vi "CommonVIs_ClassWireSelection.vi"(3 "Offset(-300,0)":T1={"Left"=-236, "Top"=18}, 4 "SaveChangesInClassRightAway(True)":bool=TRUE, 5 "WireStyleSelected":refnum<user-event>, 7 "SelectedWireStyle":refnum<vi>, 8 "error in (no error)":errorcluster, 9 "Messages(Stop or Empty string will stop this VI)":refnum<user-event>, 10 "WireSelectionList":refnum<vi>, 11 "LVClassToActOn":refnum<vi>) -> (0 "error out":errorcluster)   [LabVIEW 2020]
uses:
  Provider_BaseClassInterface/BaseProvider_SubVIs/BaseProvider_WireList.ctl
  Provider_BaseClassInterface/BaseProvider_SubVIs/BaseProvider_WireStyleType.ctl
  <vilib>/Utility/miscctls.llb/LVPositionTypeDef.ctl
  SubVIs/GOOP_WireConfigurationType.ctl
  SubVIs/GOOP_WirePattern.ctl
panel:
  out "WireEditorPresses":bool
  out "ListIndexSelected":i32
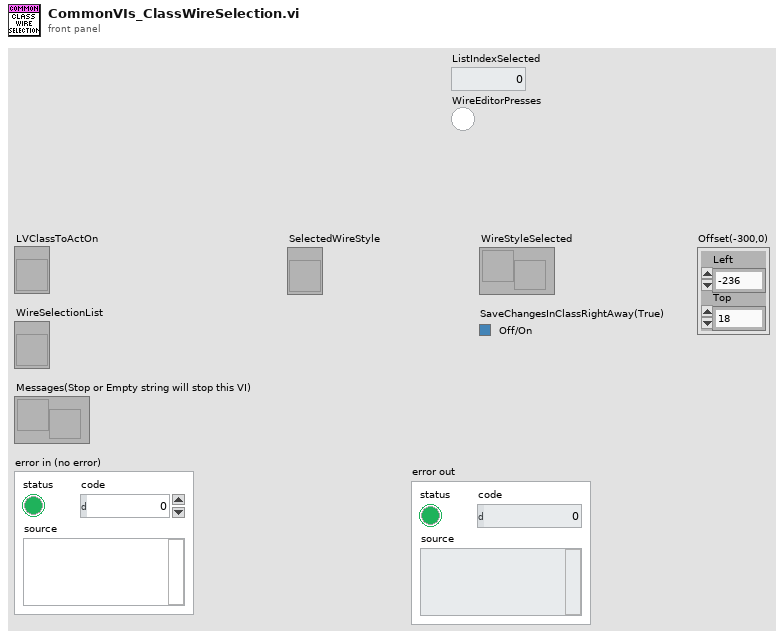
[diagram p1: front panel]
types:
  T1 = typedef "LVPositionTypeDef.ctl" = cluster{"Left":i32, "Top":i32}
  T2 = typedef "GOOP_WireConfigurationType.ctl" = cluster{"Edge thickness":i32, "Edge color":u32, "Center thickness":i32, "Center pattern":T3, "CenterColor1":u32, "CenterColor2":u32, "Tunnels and terminals colors":u32}
  T3 = typedef "GOOP_WirePattern.ctl" = enum16{"Solid", "Large dash", "Small dash"}
  T4 = typedef "BaseProvider_WireList.ctl" = cluster{"WireStyle":T5[], "WireEditor":bool}
  T5 = typedef "BaseProvider_WireStyleType.ctl" = cluster{"Boolean":bool, "Wire":picture, "Name":string, "Status":u16}
  T6 = cluster{"SelectedWireStyle":string, "Timeout":i32, "SelectedWireStyle":T2, "AllWireConfigurations(Names)":string[], "AllWireConfigurations":T2[], "SelectedWireListIndex":i32, "WireSelectionList":T4, "FirstTime":bool, "OverWireListIndex":i32, "MouseDown":bool}
  T7 = cluster{"Foreground Color":u32, "Background Color":u32, "Fill Pattern":cluster{"Row 0":u8, "Row 1":u8, "Row 2":u8, "Row 3":u8, "Row 4":u8, "Row 5":u8, "Row 6":u8, "Row 7":u8}, "Width":i16, "Mode":enum16{"Copy", "Or", "Exclusive Or", "Bit Clear", "Not Copy", "Not Or", "Nor Exclusive Or", "Not Bit Clear"}, "Style":enum32{"Solid", "Dash", "Dot", "Dash Dot", "Dash Dot Dot"}, "Fill Rule":enum32{"Even Odd", "Winding"}, "End Caps":enum32{"Default", "Flat"}}[]
  T8 = typedef "LVBoundsTypeDef.ctl" = cluster{"Width":u32, "Height":u32}
  T9 = typedef "lveventtype.ctl" = enum32{"Null", "Timeout", "Annotation Menu Selection", "Annotation Menu Selection?", "App Instance Close", "App Instance Close?", "Autoscale Range Change", "Bookmark Info Change", "Cell Edit", "Cell Edit?", "Cursor Grab", "Cursor Grab?", "Cursor Menu Selection", "Cursor Menu Selection?", "Cursor Move", "Cursor Release", "Data Change", "Direction Change", "Display State Change", "Drag Ended", "Drag Enter", "Drag Leave", "Drag Over", "Drag Source Update", "Drag Starting", "Drag Starting?", "Drop", "Exec State Change", "Key Down", "Key Down?", "Key Repeat", "Key Repeat?", "Key Up", "Listbox Double Click", "Menu Activation?", "Menu Selection (App)", "Menu Selection? (App)", "Menu Selection (User)", "Mouse Down", "Mouse Down?", "Mouse Enter", "Mouse Leave", "Mouse Move", "Mouse Up", "Mouse Wheel", "NI Security User Change (App)", "Pane Size", "Panel Close", "Panel Close?", "Panel Resize", "Plot Attribute Change", "Scale Range Change", "Shortcut Menu Activation?", "Shortcut Menu Selection (App)", "Shortcut Menu Selection? (App)", "Shortcut Menu Selection (User)", "Tree Double Click", "Tree Drag", "Tree Drag?", "Tree Drop", "Tree Drop?", "Tree Item Close", "Tree Item Close?", "Tree Item Open", "Tree Item Open?", "User Event", "Value Change"}
  T10 = typedef "LVPoint32TypeDef.ctl" = cluster{"Horizontal":i32, "Vertical":i32}
  T11 = cluster{"WireStyle":cluster{"Boolean":bool, "Wire":bool, "Name":bool, "Status":bool}[], "WireEditor":bool}
  T12 = cluster{"Boolean":bool, "Wire":bool, "Name":bool, "Status":bool}[]
  T13 = typedef "Scripting_ConnectorPanePatternType.ctl" = u16
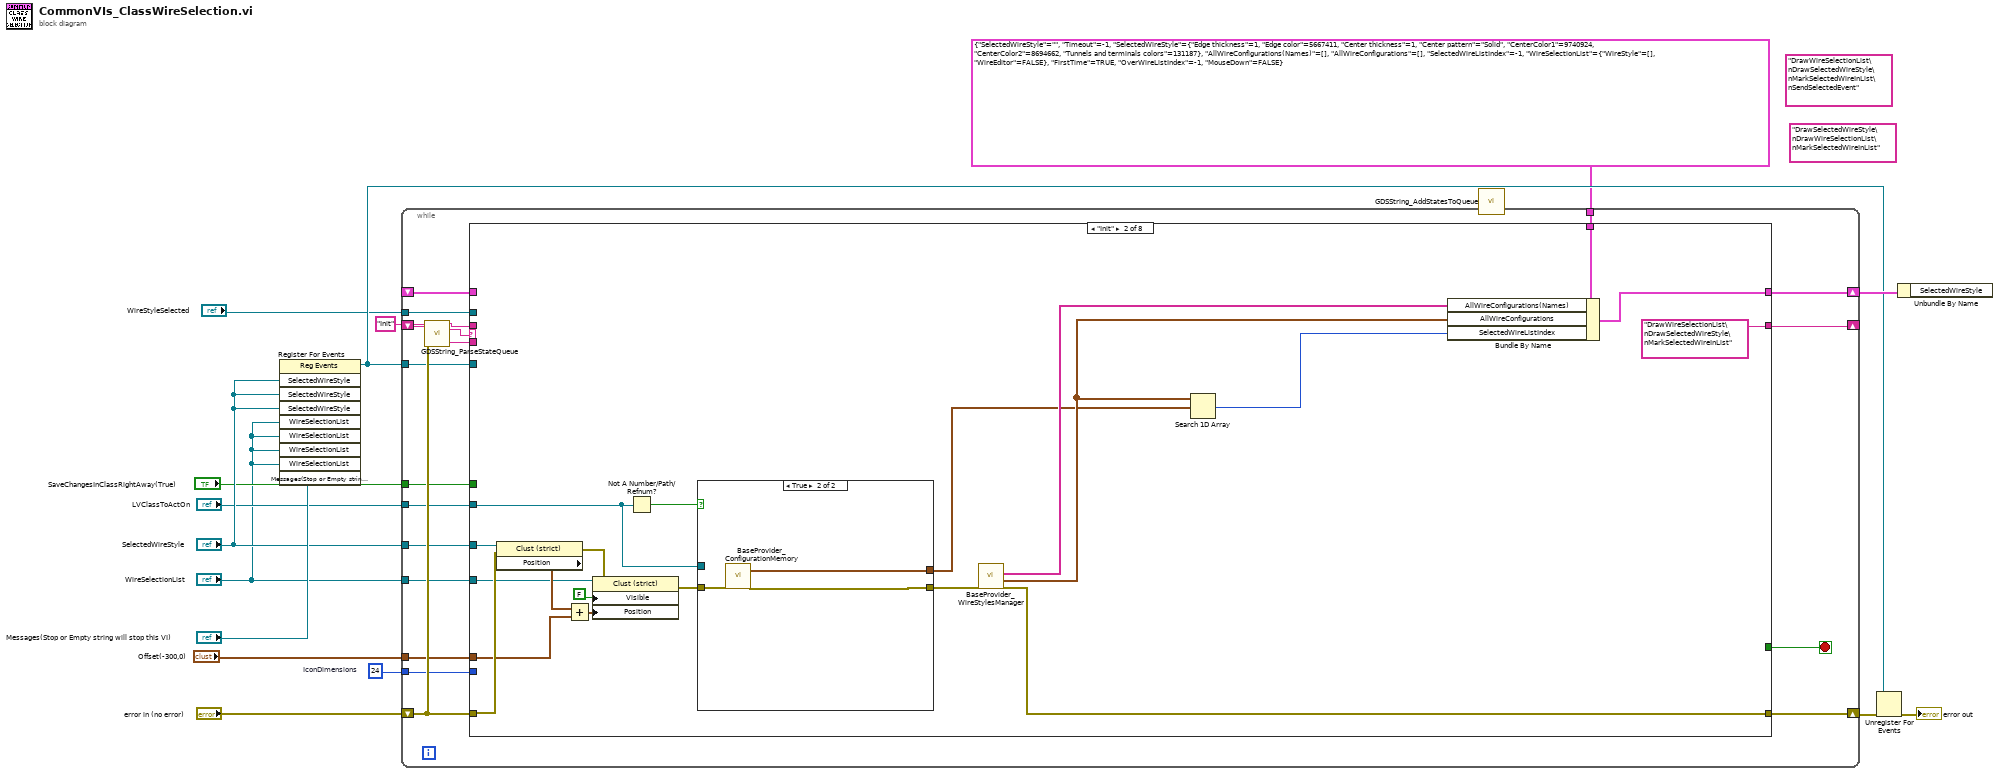
[diagram p0: block diagram]
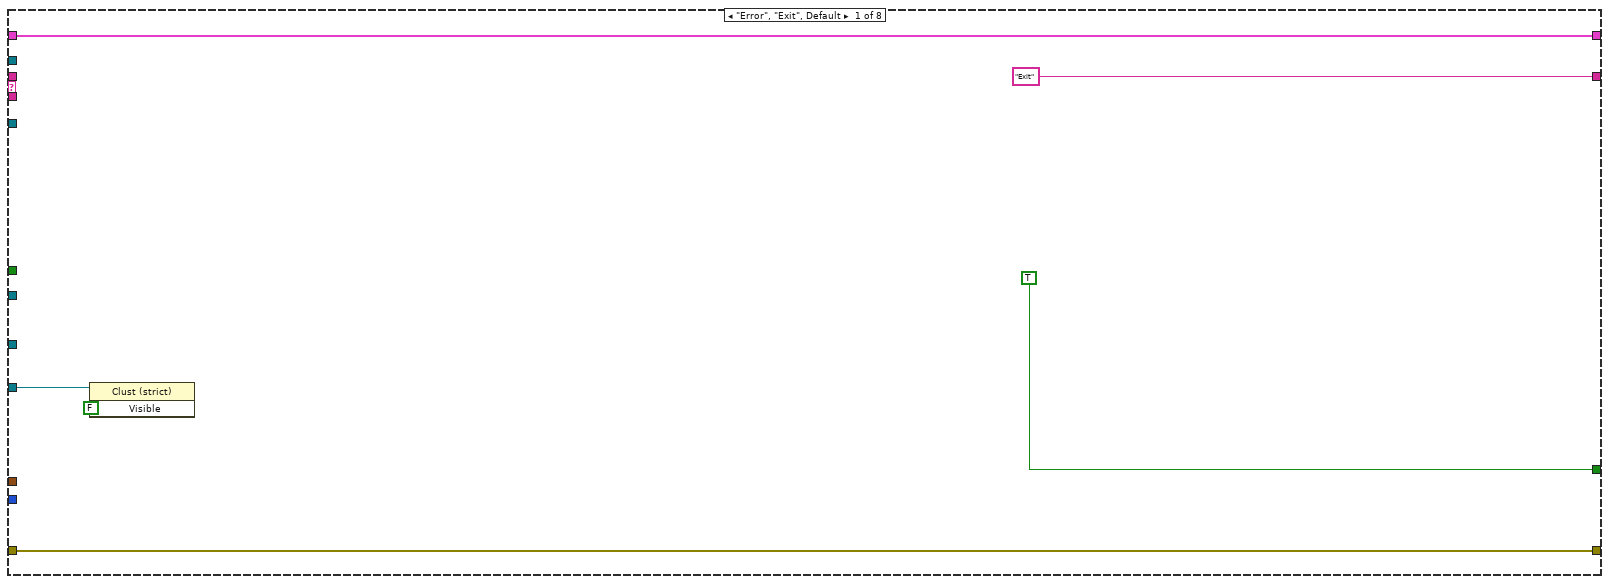
[diagram p2: hidden frame]
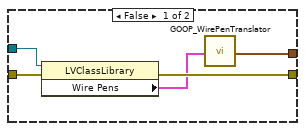
[diagram p3: hidden frame]
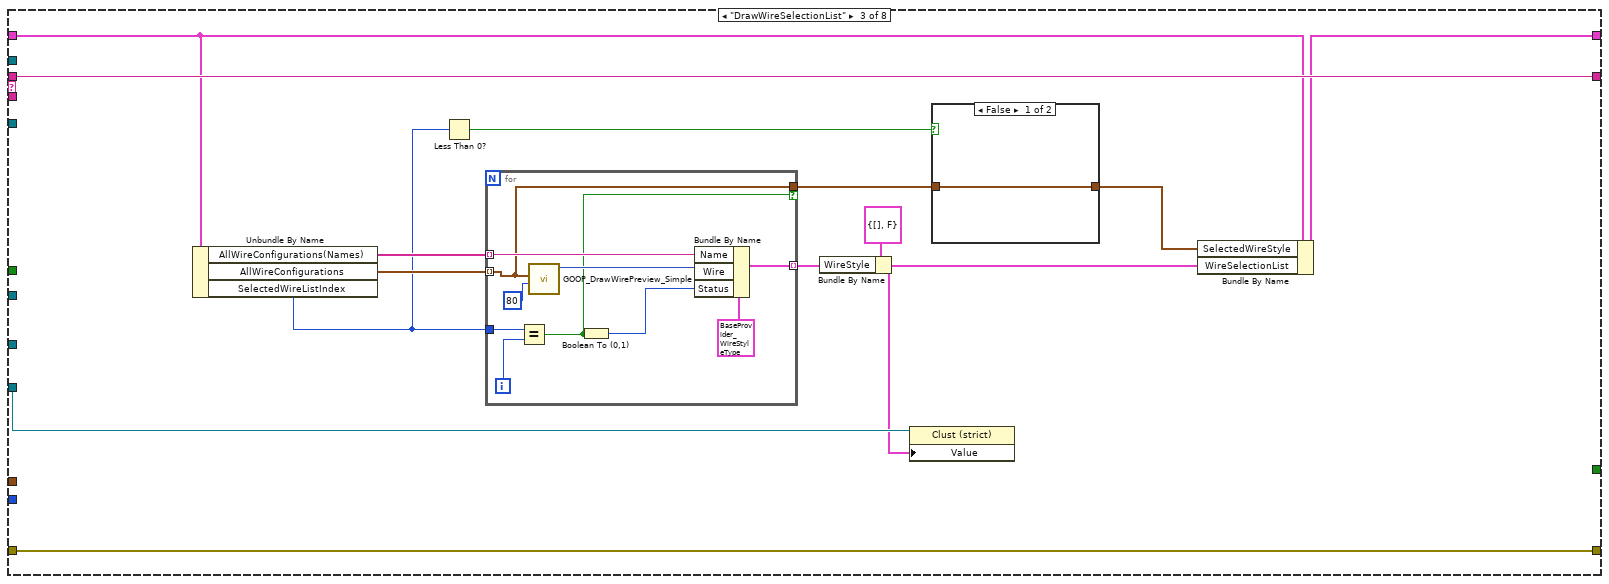
[diagram p4: hidden frame]
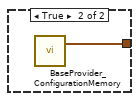
[diagram p5: hidden frame]
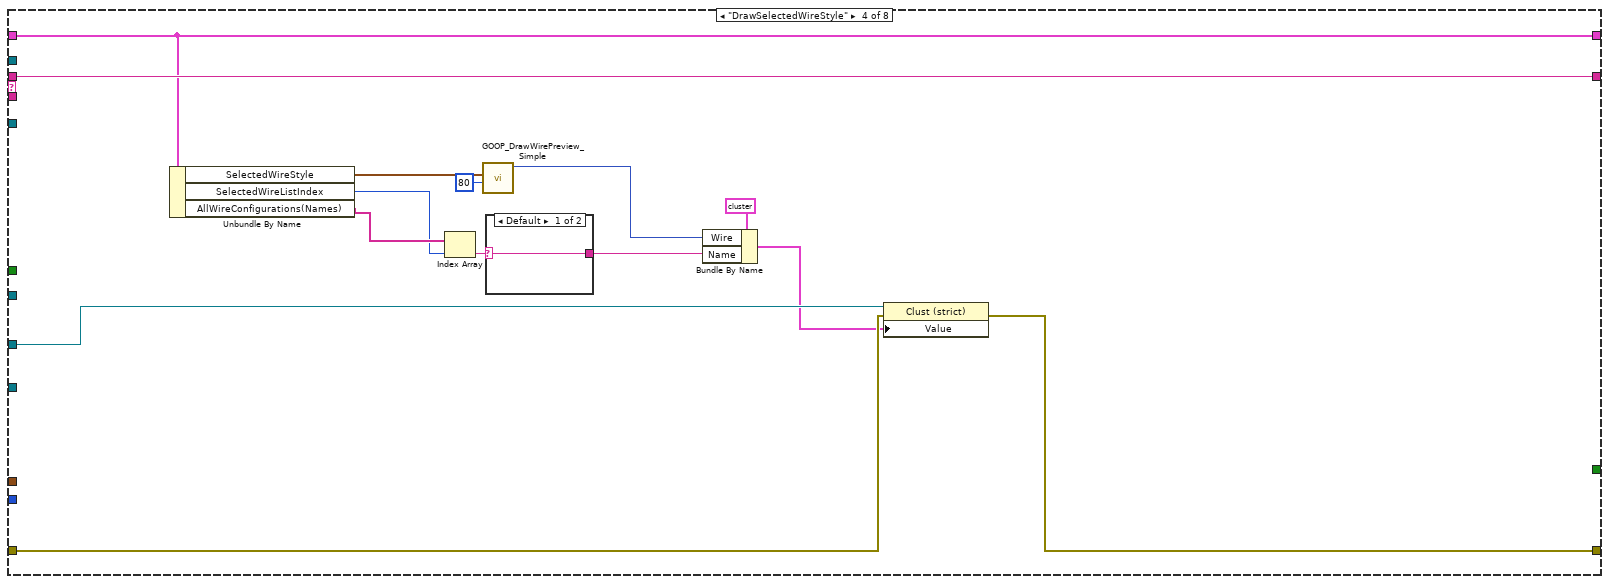
[diagram p6: hidden frame]
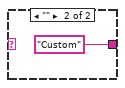
[diagram p7: hidden frame]
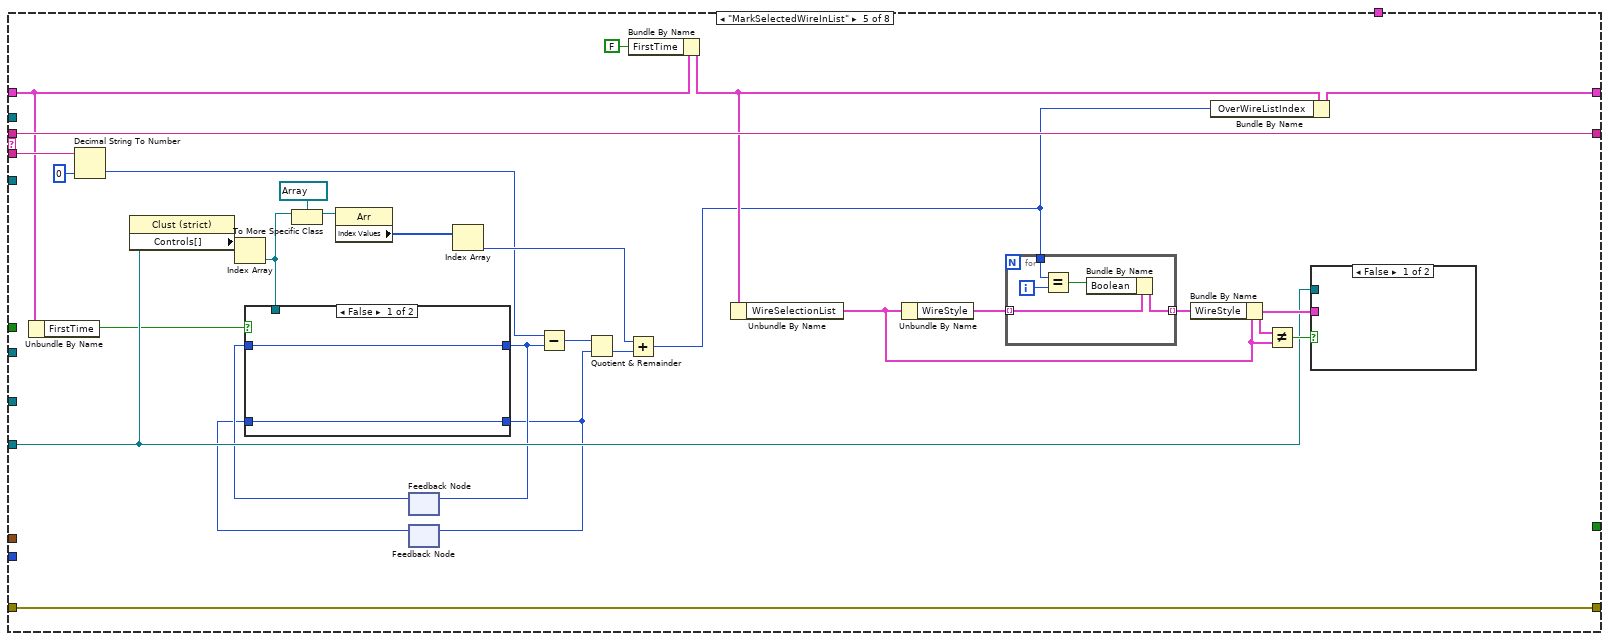
[diagram p8: hidden frame]
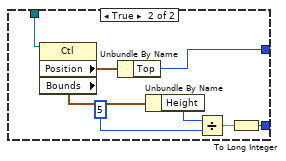
[diagram p9: hidden frame]
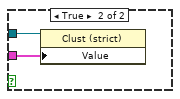
[diagram p10: hidden frame]
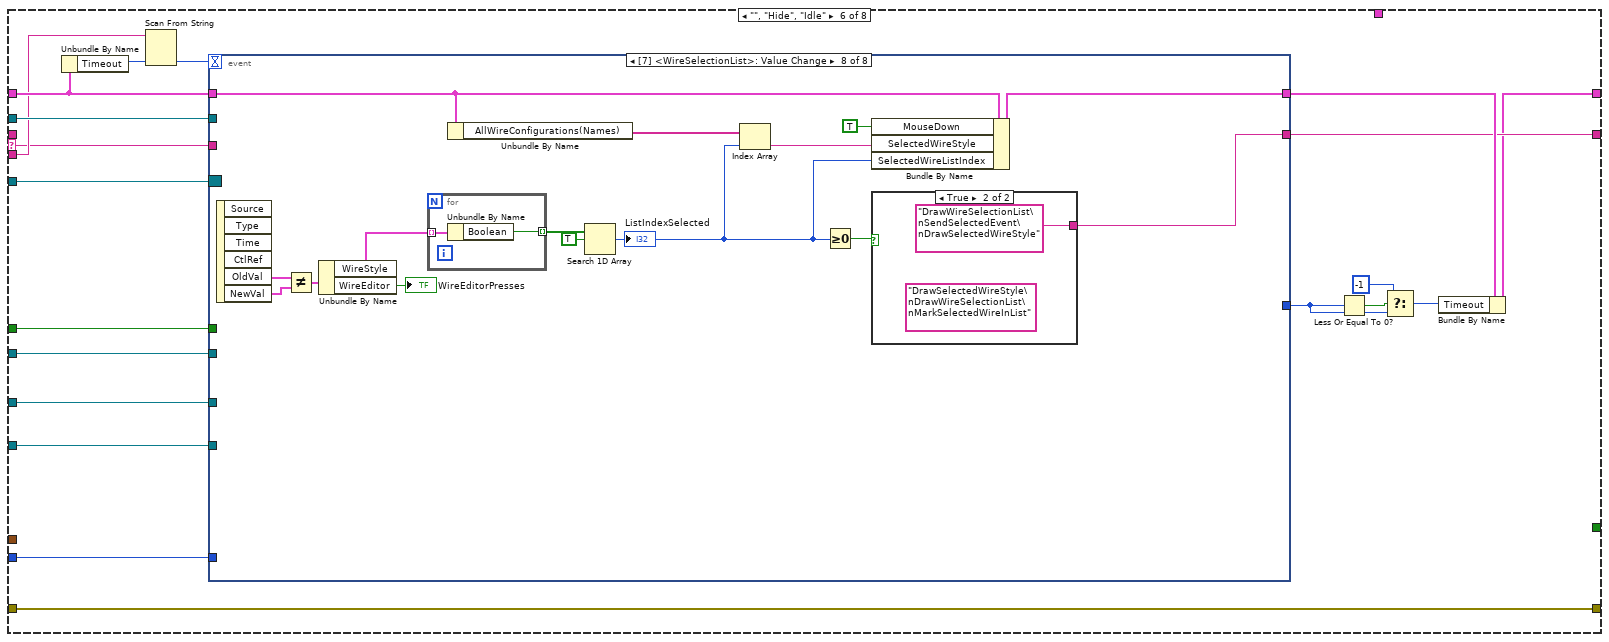
[diagram p11: hidden frame]
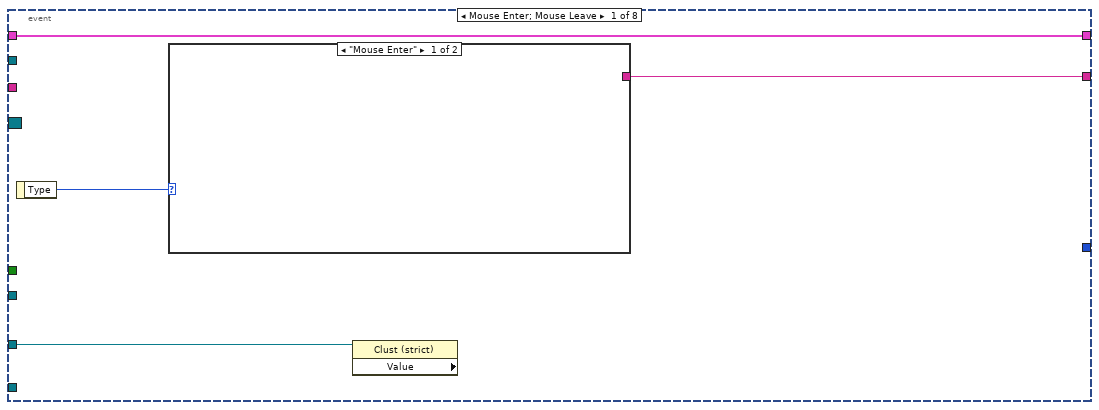
[diagram p12: hidden frame]
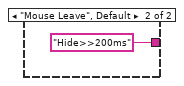
[diagram p13: hidden frame]
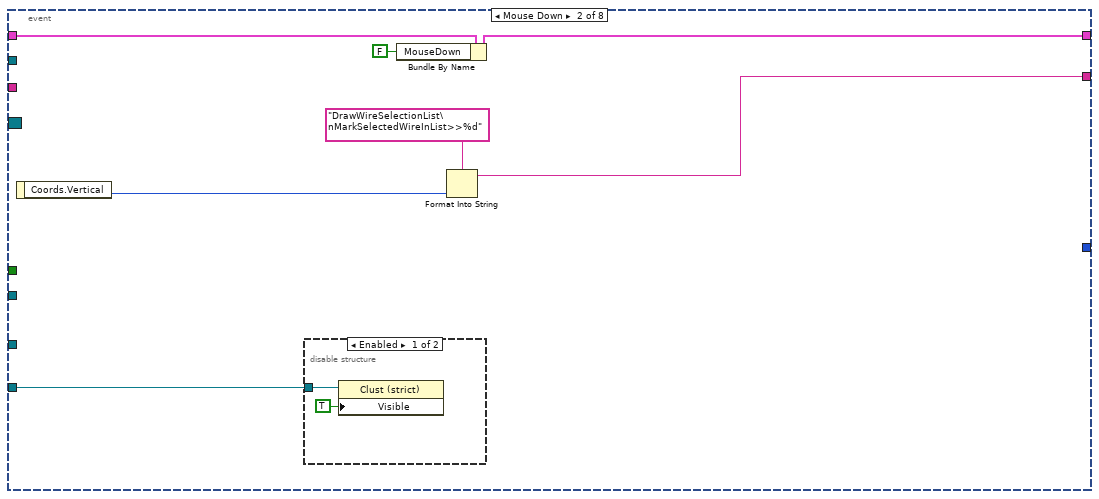
[diagram p14: hidden frame]
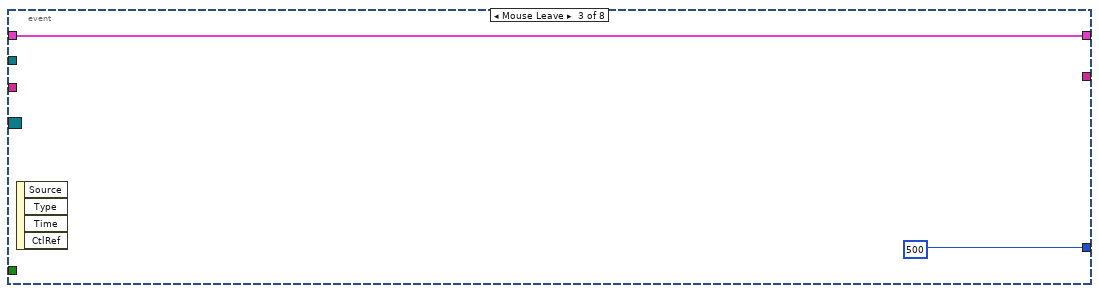
[diagram p16: hidden frame]
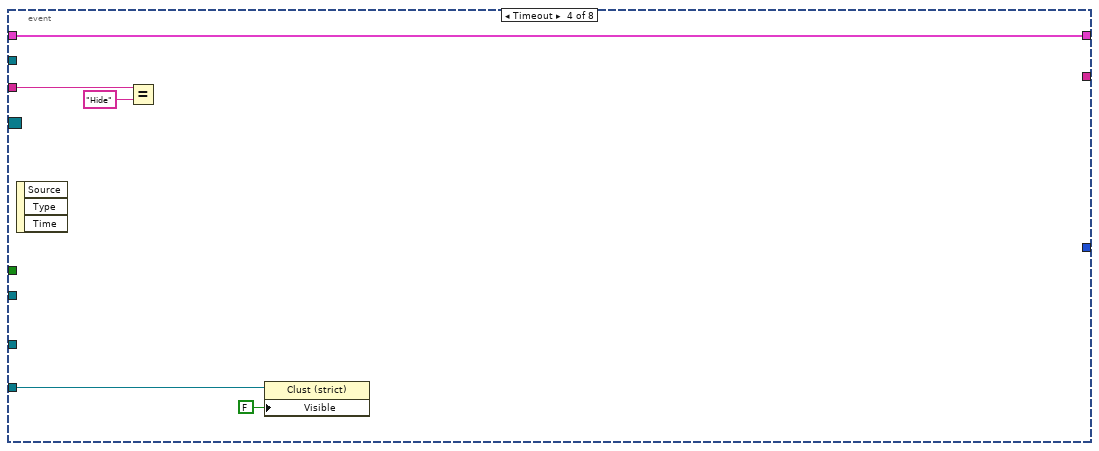
[diagram p17: hidden frame]
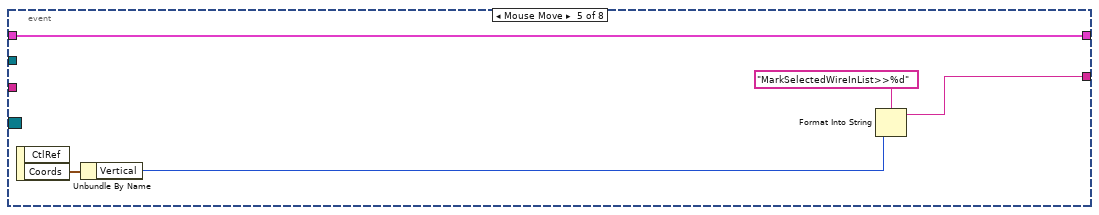
[diagram p18: hidden frame]
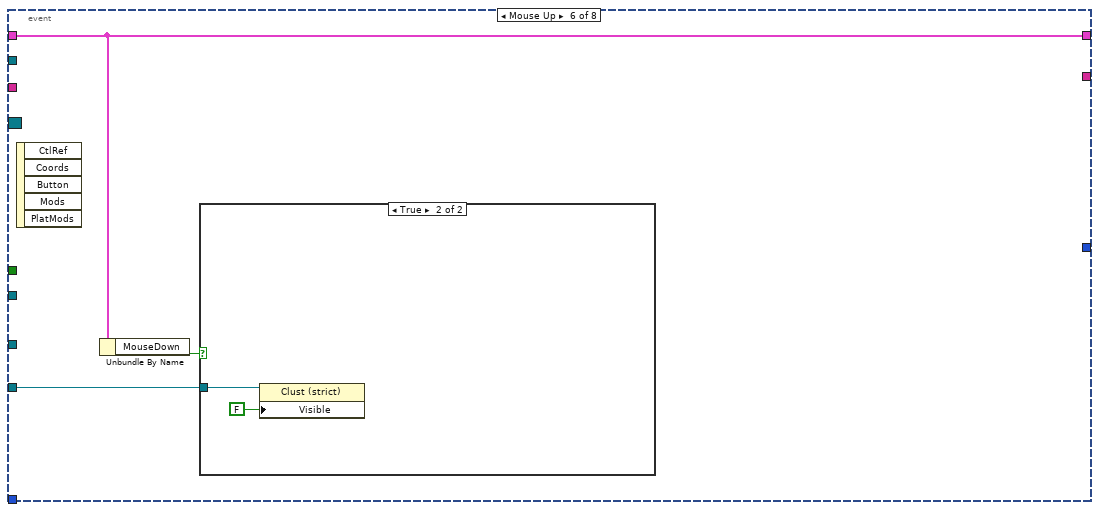
[diagram p19: hidden frame]
diagram:
  (unwired) "DrawSelectedWireStyle\nDrawWireSelectionList\nMarkSelectedWireInList"
  (unwired) "DrawWireSelectionList\nDrawSelectedWireStyle\nMarkSelectedWireInList\nSendSelectedEvent"
  w9 = i16 24  # IconDimensions
  n1 = register-events("SelectedWireStyle", "SelectedWireStyle", "SelectedWireStyle", "WireSelectionList", "WireSelectionList", "WireSelectionList", "WireSelectionList", "Messages(Stop or Empty string will stop this VI)") -> (reference out=w13:refnum<event-registration>)  [unwired: 2 in, 1 out]
  n2 = while {
    shift-right: [w30] -> w12
    shift-left: "error in (no error)" -> [w33]
    shift-right: [w29] -> _
    shift-left: "Init" -> [w34]
    tunnel: "WireSelectionList" -> [w32]
    tunnel: "SelectedWireStyle" -> [w31]
    tunnel: w9 -> [w25]
    tunnel: T6 {"SelectedWireStyle"="", "Timeout"=-1, "SelectedWireStyle"={"Edge thickness"=1, "Edge color"=5667411, "Center thickness"=1, "Center pattern"=enum."Solid", "CenterColor1"=9740924, "CenterColor2"=8694662, "Tunnels and terminals colors"=131187}, "AllWireConfigurations(Names)"=[], "AllWireConfigurations"=[], "SelectedWireListIndex"=-1, "WireSelectionList"={"WireStyle"=[], "WireEditor"=FALSE}, "FirstTime"=TRUE, "OverWireListIndex"=-1, "MouseDown"=FALSE} -> [w24]
    shift-right: [w23] -> w14
    shift-left: _ -> [w22]
    tunnel: w13 -> [w21]
    tunnel: "LVClassToActOn" -> [w20]
    tunnel: "WireStyleSelected" -> [w19]
    tunnel: "SaveChangesInClassRightAway(True)" -> [w18]
    tunnel: "Offset(-300,0)" -> [w17]
    stop <- w28 stop-if-true
    n3 = call "GDSString_ParseStateQueue.vi"("State Queue"=w34, "Error In (no error)"=w33) -> ("Remaining States"=w27:string, "Current State"=w26:string, "Arguments"=w16:string)  [unwired: 9 in, 2 out]
    n4 = case shown="\"Init\"" w26 {
      selector: w26 -> [_ _ _ _ _ w157 _ _]
      tunnel: w33 -> [w40 w58 w82 w105 w138 w176 w244 w257]
      tunnel: w32 -> [w36 w52 w80 _ w123 w172 _ _]
      tunnel: w31 -> [_ w53 _ w106 _ w164 _ _]
      tunnel: [w40 w45 w82 w108 w138 w176 w242 w257] -> w30
      tunnel: ["Exit" "DrawWireSelectionList\nDrawSelectedWireStyle\nMarkSelectedWireInList" w81 w107 w139 w173 w237 w256] -> w29
      tunnel: [TRUE _ _ _ _ _ _ _] -> w28
      tunnel: w27 -> [_ _ w81 w107 w139 _ w239 w256]
      tunnel: w25 -> [_ _ _ _ _ w171 _ _]
      tunnel: w24 -> [_ w55 _ _ _ _ _ _]
      tunnel: [w37 w54 w74 w95 w112 w170 w243 w254] -> w23
      tunnel: w22 -> [w37 _ w79 w95 w116 w165 w246 w254]
      tunnel: w21 -> [_ _ _ _ _ w175 _ _]
      tunnel: w20 -> [_ w50 _ _ _ w163 _ _]
      tunnel: w19 -> [_ _ _ _ _ w162 _ w255]
      tunnel: w18 -> [_ _ _ _ _ w161 _ _]
      tunnel: w17 -> [_ w47 _ _ _ _ _ _]
      tunnel: w16 -> [_ _ _ _ w132 w160 _ _]
      frame "Error", "Exit", Default {
        n5 = property class="Clust (strict)"(reference=w36, "Visible"=FALSE) -> ()  [unwired: 1 in, 2 out]
      }
      frame "Init" {
        n6 = property class="Clust (strict)"(reference=w53, error in=w58) -> (error out=w57:errorcluster, "Position"=w60:T1)  [unwired: 1 out]
        n7 = Add(x=w60, y=w47) -> (x+y=w48:T1)
        n8 = property class="Clust (strict)"(reference=w52, error in=w57, "Visible"=FALSE, "Position"=w48) -> (error out=w56:errorcluster)  [unwired: 1 out]
        n9 = Not A Number/Path/Refnum?(number/path/refnum=w50) -> (NaN/Path/Refnum?=w51:bool)
        n10 = case shown="True" w51 {
          tunnel: w56 -> [w64 w68]
          tunnel: [w63 w67] -> w46
          tunnel: [w62 w66] -> w42
          tunnel: w50 -> [w65 _]
          frame False {
            n11 = property class="LVClassLibrary"(reference=w65, error in=w64) -> (error out=w63:errorcluster, "Wire Pens"=w61:T7)  [unwired: 1 out]
            n12 = call "GOOP_WirePenTranslator.vi"("WirePensIn"=w61) -> ("WireConfigurationOut"=w62:T2)  [unwired: 17 in, 1 out]
          }
          frame True {
            n13 = call "BaseProvider_ConfigurationMemory.vi"("error in (no error)"=w68) -> ("WireConfigurationOut"=w66:T2, "error out"=w67:errorcluster)  [unwired: 12 in, 5 out]
          }
        }
        n14 = call "BaseProvider_WireStylesManager.vi"("error in (no error)"=w46) -> ("error out"=w45:errorcluster, "AllWireConfigurations"=w43:T2[], "AllWireConfigurations(Names)"=w44:string[])  [unwired: 7 in, 1 out]
        n15 = Search 1D Array(1D array=w43, element=w42) -> (index of element=w41:i32)  [unwired: 1 in]
        n16 = Bundle By Name(cluster=w55, "AllWireConfigurations(Names)"=w44, "AllWireConfigurations"=w43, "SelectedWireListIndex"=w41) -> (w54:T6)
      }
      frame "DrawWireSelectionList" {
        n17 = Unbundle By Name(w79) -> ("AllWireConfigurations(Names)"=w78:string[], "AllWireConfigurations"=w77:T2[], "SelectedWireListIndex"=w72:i32)
        n18 = Less Than 0?(x=w72) -> (x < 0?=w71:bool)
        n19 = for {
          tunnel: w78 -> [w94] mode=indexing
          tunnel: w77 -> [w86] mode=indexing
          tunnel: w72 -> [w90]
          tunnel: [w89] -> w75 mode=indexing
          tunnel: [w86] -> w70 if=w85
          i -> [w91]
          n20 = Equal?(x=w90, y=w91) -> (x = y?=w85:bool)
          n21 = call "GOOP_DrawWirePreview_Simple.vi"("WireLength(100px)"=i16 80, "WireConfiguration"=w86) -> ("WirePictureOut"=w92:picture)  [unwired: 5 in, 4 out]
          n22 = Boolean To (0,1)(Boolean=w85) -> (0, 1=w88:i16)
          n23 = Bundle By Name(cluster=T5 {"Boolean"=FALSE, "Wire"=bytes[0], "Name"="", "Status"=0} ("Cluster 2"), "Name"=w94, "Wire"=w92, "Status"=w88) -> (w89:T5)
        }
        n24 = Bundle By Name(cluster=T4 {"WireStyle"=[], "WireEditor"=FALSE} ("WireSelectionList 2"), "WireStyle"=w75) -> (w73:T4)
        n25 = property class="Clust (strict)"(reference=w80, "Value"=w73) -> ()  [unwired: 1 in, 2 out]
        n26 = case shown="False" w71 {
          tunnel: w70 -> [w83 _]
          tunnel: [w83 w84] -> w69
          frame False {
          }
          frame True {
            n27 = call "BaseProvider_ConfigurationMemory.vi"() -> ("WireConfigurationOut"=w84:T2)  [unwired: 13 in, 6 out]
          }
        }
        n28 = Bundle By Name(cluster=w79, "SelectedWireStyle"=w69, "WireSelectionList"=w73) -> (w74:T6)
      }
      frame "DrawSelectedWireStyle" {
        n29 = Unbundle By Name(w95) -> ("SelectedWireStyle"=w99:T2, "SelectedWireListIndex"=w96:i32, "AllWireConfigurations(Names)"=w100:string[])
        n30 = Index Array(array=w100, index=w96) -> (element=w98:string)
        n31 = call "GOOP_DrawWirePreview_Simple.vi"("WireLength(100px)"=i16 80, "WireConfiguration"=w99) -> ("WirePictureOut"=w102:picture)  [unwired: 5 in, 4 out]
        n32 = case shown="Default" w98 {
          selector: w98 -> [w109 _]
          tunnel: [w109 "Custom"] -> w97
          frame Default {
          }
          frame "" {
          }
        }
        n33 = Bundle By Name(cluster=cluster{"Name":string, "Wire":picture} {"Name"="Default", "Wire"=bytes[0]} ("Value"), "Wire"=w102, "Name"=w97) -> (w103:cluster{"Name":string, "Wire":picture})
        n34 = property class="Clust (strict)"(reference=w106, error in=w105, "Value"=w103) -> (error out=w108:errorcluster)  [unwired: 1 out]
      }
      frame "MarkSelectedWireInList" {
        n35 = Unbundle By Name(w116) -> ("FirstTime"=w115:bool)
        n36 = Decimal String To Number(string=w132, default (0L)=0 ("default (0 I32)")) -> (number=w124:i32)  [unwired: 1 in, 1 out]
        n37 = property class="Clust (strict)"(reference=w123) -> ("Controls[]"=w130:refnum<vi>[])  [unwired: 1 in, 2 out]
        n38 = Index Array(array=w130) -> (element=w119:refnum<vi>)  [unwired: 1 in]
        n39 = To More Specific Class(target class=refnum<vi> refnum ("reference"), reference=w119) -> (specific class reference=w129:refnum<vi>)  [unwired: 1 in, 1 out]
        n40 = property class="Arr"(reference=w129) -> ("Index Values"=w128:u32[])  [unwired: 1 in, 2 out]
        n41 = feedback #1() -> (w114:i32)  [unwired: 1 in]
        n42 = feedback #2() -> (w113:i32)  [unwired: 1 in]
        n43 = case shown="False" w115 {
          tunnel: w119 -> [_ w144]
          tunnel: [w141 w143] -> w118
          tunnel: [w140 w142] -> w117
          tunnel: w114 -> [w141 _]
          tunnel: w113 -> [w140 _]
          frame False {
          }
          frame True {
            n44 = property class="Ctl"(reference=w144) -> ("Position"=w147:T1, "Bounds"=w145:T8)  [unwired: 1 in, 2 out]
            n45 = Unbundle By Name(w147) -> ("Top"=w143:i32)
            n46 = Unbundle By Name(w145) -> ("Height"=w149:u32)
            n47 = Divide(x=w149, y=u32 5) -> (x/y=w148:dbl)
            n48 = To Long Integer(number=w148) -> (32bit integer=w142:i32)
          }
        }
        n49 = feedback-in #1(w118) -> ()
        n50 = feedback-in #2(w117) -> ()
        n51 = Index Array(array=w128) -> (element=w127:u32)  [unwired: 1 in]
        n52 = Subtract(x=w124, y=w118) -> (x-y=w125:i32)
        n53 = Quotient & Remainder(x=w125, y=w117) -> (floor(x/y)=w126:i32)  [unwired: 1 out]
        n54 = Add(x=w127, y=w126) -> (x+y=w111:u32)
        n55 = Bundle By Name(cluster=w116, "FirstTime"=FALSE) -> (w122:T6)
        n56 = Unbundle By Name(w122) -> ("WireSelectionList"=w133:T4)
        n57 = Unbundle By Name(w133) -> ("WireStyle"=w134:T5[])
        n58 = for {
          tunnel: w134 -> [w154] mode=indexing
          tunnel: w111 -> [w155]
          tunnel: [w152] -> w137 mode=indexing
          i -> [w156]
          n59 = Equal?(x=w155, y=w156) -> (x = y?=w153:bool)
          n60 = Bundle By Name(cluster=w154, "Boolean"=w153) -> (w152:T5)
        }
        n61 = Bundle By Name(cluster=w133, "WireStyle"=w137) -> (w135:T4)
        n62 = Bundle By Name(cluster=w122, "OverWireListIndex"=w111) -> (w112:T6)
        n63 = Not Equal?(x=w135, y=w133) -> (x != y?=w136:bool)
        n64 = case shown="False" w136 {
          tunnel: w123 -> [_ w151]
          tunnel: w135 -> [_ w150]
          frame False {
          }
          frame True {
            n65 = property class="Clust (strict)"(reference=w151, "Value"=w150) -> ()  [unwired: 1 in, 2 out]
          }
        }
      }
      frame "", "Hide", "Idle" {
        n66 = Unbundle By Name(w165) -> ("Timeout"=w159:i32)
        n67 = Scan From String(input string=w160, default 1=w159) -> (output 1=w158:i32)  [unwired: 3 in, 3 out]
        n68 = event shown="[7] <WireSelectionList>: Value Change" {
          selector: w175 -> [_ _ _ _ _ _ _ _]
          dyn-events: _ -> [_ _ _ _ _ _ _ _]
          timeout: w158 -> [_ _ _ _ _ _ _ _]
          tunnel: w165 -> [w179 w185 w192 w197 w202 w203 w208 w219]
          tunnel: [w179 w184 w192 w197 w202 w203 w209 w222] -> w174
          tunnel: [w177 w186 _ _ w200 _ w210 w215] -> w173
          tunnel: w172 -> [_ w188 _ w196 _ w205 _ _]
          tunnel: w171 -> [_ _ _ _ _ _ _ _]
          tunnel: [_ _ 500 ("500") _ _ _ _ _] -> w167
          tunnel: w164 -> [w178 _ _ _ _ _ _ _]
          tunnel: w163 -> [_ _ _ _ _ _ _ _]
          tunnel: w162 -> [_ _ _ _ _ _ _ _]
          tunnel: w161 -> [_ _ _ _ _ _ _ _]
          tunnel: w157 -> [_ _ _ w195 _ _ _ _]
          event Mouse Enter; Mouse Leave {
            n69 = event-data() -> ("Type"=w180:T9)  [unwired: 1 in]
            n70 = case shown="\"Mouse Enter\"" w180 {
              tunnel: [_ "Hide>>200ms"] -> w177
              frame "Mouse Enter" {
              }
              frame "Mouse Leave", Default {
              }
            }
            n71 = property class="Clust (strict)" props=["Value"](reference=w178) -> ()  [unwired: 1 in, 3 out]
          }
          event Mouse Down {
            n72 = event-data() -> ("Coords.Vertical"=w187:i32)  [unwired: 1 in]
            n73 = disable-structure shown="Enabled" {
              disable-tunnel: w188 -> [w190 _]
              frame Enabled {
                n74 = property class="Clust (strict)"(reference=w190, "Visible"=TRUE) -> ()  [unwired: 1 in, 2 out]
              }
              frame Disabled {
              }
            }
            n75 = Bundle By Name(cluster=w185, "MouseDown"=FALSE) -> (w184:T6)
            n76 = Format Into String(format string="DrawWireSelectionList\nMarkSelectedWireInList>>%d", w187) -> (resulting string=w186:string)  [unwired: 2 in, 1 out]
          }
          event Mouse Leave {
            n77 = event-data() -> ()  [unwired: 1 in, 4 out]
          }
          event Timeout {
            n78 = event-data() -> ()  [unwired: 1 in, 3 out]
            n79 = Equal?(x=w195, y="Hide") -> ()  [unwired: 1 out]
            n80 = property class="Clust (strict)"(reference=w196, "Visible"=FALSE) -> ()  [unwired: 1 in, 2 out]
          }
          event Mouse Move {
            n81 = event-data() -> ("Coords"=w199:T10)  [unwired: 1 in, 1 out]
            n82 = Unbundle By Name(w199) -> ("Vertical"=w198:i32)
            n83 = Format Into String(format string="MarkSelectedWireInList>>%d", w198) -> (resulting string=w200:string)  [unwired: 2 in, 1 out]
          }
          event Mouse Up {
            n84 = event-data() -> ()  [unwired: 1 in, 5 out]
            n85 = Unbundle By Name(w203) -> ("MouseDown"=w204:bool)
            n86 = case shown="True" w204 {
              tunnel: w205 -> [_ w206]
              frame False {
              }
              frame True {
                n87 = property class="Clust (strict)"(reference=w206, "Visible"=FALSE) -> ()  [unwired: 1 in, 2 out]
              }
            }
          }
          event User Event {
            n88 = event-data() -> ("Stop"=w211:string)  [unwired: 1 in, 4 out]
            n89 = case shown="\"\", \"stop\"" w211 {
              tunnel: [_ "Exit"] -> w210
              tunnel: w208 -> [w212 w213]
              tunnel: [w212 w213] -> w209
              tunnel: w208 -> [_ _]
              frame Default {
              }
              frame "", "stop" {
              }
            }
          }
          event Value Change {
            n90 = event-data() -> ("OldVal"=w229:T4, "NewVal"=w228:T4)  [unwired: 1 in, 4 out]
            n91 = Not Equal?(x=w229, y=w228) -> (x != y?=w227:T11)
            n92 = Unbundle By Name(w227) -> ("WireStyle"=w226:T12, "WireEditor"=→"WireEditorPresses":bool)
            n93 = for {
              tunnel: w226 -> [w233] mode=indexing
              tunnel: [w232] -> w225 mode=indexing
              n94 = Unbundle By Name(w233) -> ("Boolean"=w232:bool)
            }
            n95 = Unbundle By Name(w219) -> ("AllWireConfigurations(Names)"=w218:string[])
            n96 = Search 1D Array(1D array=w225, element=TRUE) -> (index of element=w217:i32)  [unwired: 1 in]
            "ListIndexSelected" <- w217
            n97 = Index Array(array=w218, index=w217) -> (element=w216:string)
            n98 = Greater Or Equal To 0?(x=w217) -> (x >= 0?=w220:bool)
            n99 = Bundle By Name(cluster=w219, "MouseDown"=TRUE, "SelectedWireStyle"=w216, "SelectedWireListIndex"=w217) -> (w222:T6)
            n100 = case shown="True" w220 {
              tunnel: ["OpenWireStyleEditor" "DrawWireSelectionList\nSendSelectedEvent\nDrawSelectedWireStyle"] -> w215
              frame False {
              }
              frame True {
                (unwired) "DrawSelectedWireStyle\nDrawWireSelectionList\nMarkSelectedWireInList"
              }
            }
          }
        }
        n101 = Less Or Equal To 0?(x=w167) -> (x <= 0?=w169:bool)
        n102 = Select(t=-1, s=w169, f=w167) -> (s? t:f=w168:i32)
        n103 = Bundle By Name(cluster=w174, "Timeout"=w168) -> (w170:T6)
      }
      frame "OpenWireStyleEditor" {
        n104 = call "BaseProvider_Configuration.vi"("OnlyWireStyleConfiguration(False)"=TRUE, "Error In"=w244) -> ("SelectedWireStyleIndex"=w240:i32, "Error Out"=w234:errorcluster)  [unwired: 16 in]
        n105 = call "BaseProvider_WireStylesManager.vi"("error in (no error)"=w234) -> ("error out"=w242:errorcluster, "AllWireConfigurations"=w235:T2[], "AllWireConfigurations(Names)"=w236:string[])  [unwired: 7 in, 1 out]
        n106 = case shown="0, Default" w240 {
          selector: w240 -> [w248 _]
          tunnel: [w249 "Custom" ("String")] -> w241
          tunnel: w236 -> [w247 _]
          frame 0, Default {
            n107 = Index Array(array=w247, index=w248) -> (element=w249:string)
          }
          frame -1 {
          }
        }
        n108 = Bundle By Name(cluster=w246, "SelectedWireStyle"=w241, "SelectedWireListIndex"=w240, "AllWireConfigurations(Names)"=w236, "AllWireConfigurations"=w235) -> (w243:T6)
        n109 = call "GDSString_AddStatesToQueue.vi"("State(s) in (\"\")"=w239, "State(s) at Back (\"\")"="DrawWireSelectionList\nDrawSelectedWireStyle\nMarkSelectedWireInList\nSendSelectedEvent") -> ("States Out"=w237:string)  [unwired: 13 in]
      }
      frame "SendSelectedEvent" {
        n110 = Unbundle By Name(w254) -> ("SelectedWireStyle"=w253:string, "AllWireConfigurations"=w252:T2[], "SelectedWireListIndex"=w251:i32)
        n111 = case shown="-1" w251 {
          selector: w251 -> [w262 _]
          tunnel: w252 -> [w263 _]
          frame 0, Default {
            n112 = call "BaseProvider_ConfigurationMemory.vi"() -> ("PatternOut"=w258:T13, "IconOut"=w259:string)  [unwired: 13 in, 5 out]
            n113 = Index Array(array=w263, index=w262) -> (element=w261:T2)
            n114 = call "BaseProvider_ConfigurationMemory.vi"("WireConfiguration"=w261, "Icon"=w259, "Action"=enum16{"Read", "Load", "Save", "Set"}."Save", "PatternIn"=w258) -> ()  [unwired: 9 in, 7 out]
          }
          frame -1 {
          }
        }
        n115 = Generate User Event(user event=w255, event data cluster=w253) -> ()  [unwired: 2 in, 2 out]
      }
    }
  }
  n116 = call "GDSString_AddStatesToQueue.vi"() -> ()  [unwired: 15 in, 1 out]
  n117 = Unregister For Events(event registration refnum=w13, error in=w12) -> (error out=→"error out":errorcluster)
  n118 = Unbundle By Name(w14) -> ()  [unwired: 1 out]
